vi "C_Info.vi"(8 "error in (no error)":errorcluster) -> (0 "error out":errorcluster, 3 "C_Info":T1)   [LabVIEW 2021, in "CANsub_C.lvlib"]
uses:
  CANsub_C.lvlib
  codec_vis/CANsub_Codec.lvlib
  C_Info.ctl
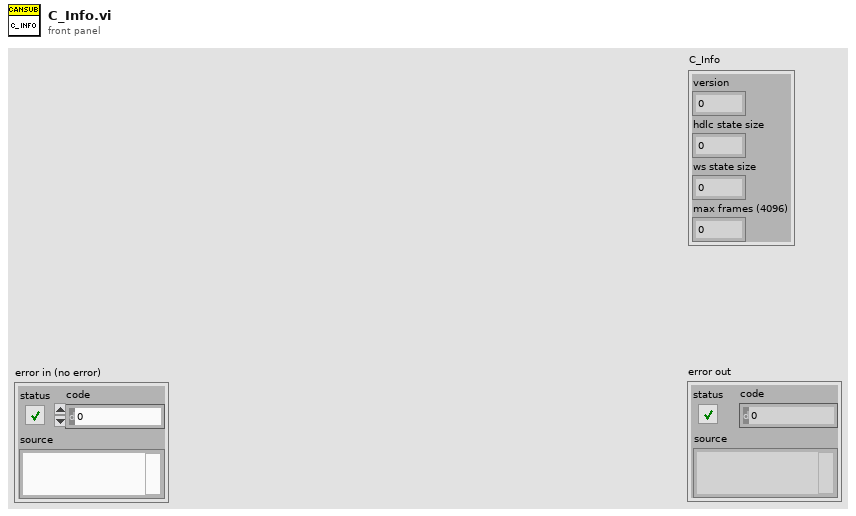
[diagram p1: front panel]
types:
  T1 = typedef "CANsub_C.lvlib/C_Info.ctl" = cluster{"version":u32, "hdlc state size":i32, "ws state size":i32, "max frames (4096)":i32}
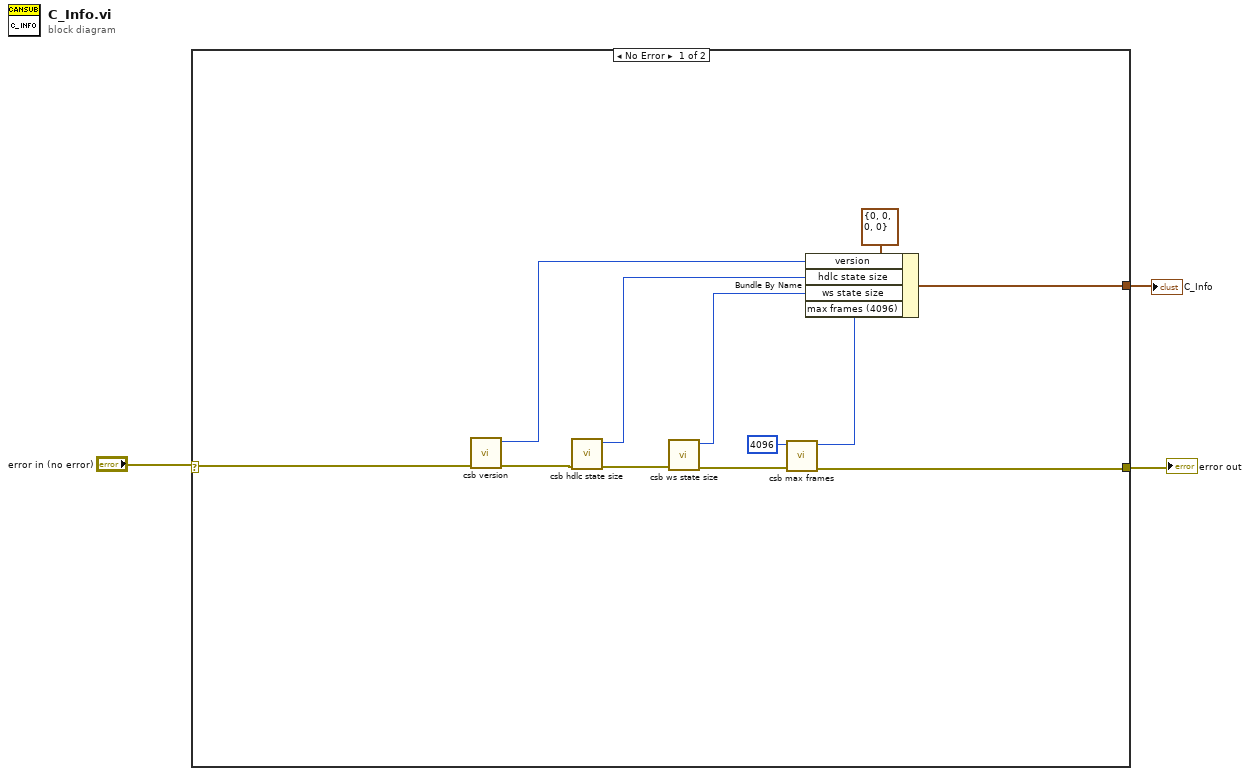
[diagram p0: block diagram]
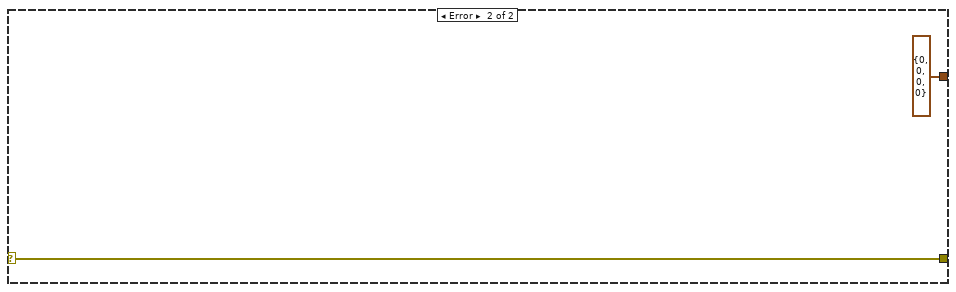
[diagram p2: hidden frame]
diagram:
  n1 = case shown="No Error" "error in (no error)" {
    selector: "error in (no error)" -> [w14 w17]
    tunnel: [w10 w17] -> w2
    tunnel: [w4 T1 {"version"=0, "hdlc state size"=0, "ws state size"=0, "max frames (4096)"=0} ("C_Info")] -> w1
    frame No Error {
      n2 = call "csb version.vi"("error in (no error)"=w14) -> ("error out"=w13:errorcluster, "function return"=w8:u32)  [unwired: 9 in]
      n3 = call "csb hdlc state size.vi"("error in (no error)"=w13) -> ("error out"=w12:errorcluster, "function return"=w7:i32)  [unwired: 9 in]
      n4 = call "csb ws state size.vi"("error in (no error)"=w12) -> ("error out"=w11:errorcluster, "function return"=w6:i32)  [unwired: 9 in]
      n5 = call "csb max frames.vi"("error in (no error)"=w11, "in_len"=4096) -> ("error out"=w10:errorcluster, "function return"=w5:i32)  [unwired: 8 in]
      n6 = Bundle By Name(cluster=T1 {"version"=0, "hdlc state size"=0, "ws state size"=0, "max frames (4096)"=0} ("C_Info"), "version"=w8, "hdlc state size"=w7, "ws state size"=w6, "max frames (4096)"=w5) -> (w4:T1)
    }
    frame Error {
    }
  }
  "error out" <- w2
  "C_Info" <- w1
